vi "Type Definition Folder Name--constant.vi"() -> (3 "Type Definition Folder Name":string)   [LabVIEW 2026]
doc: "This constant defines the name of the type definitions folder on the main project directory."
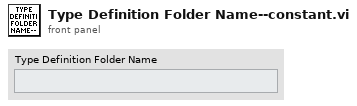
[diagram p1: front panel]
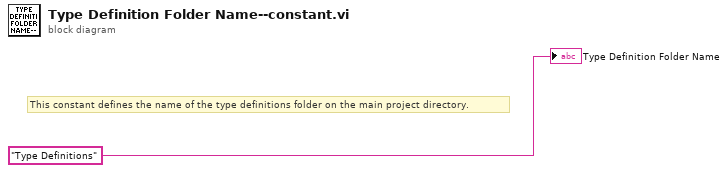
[diagram p0: block diagram]
diagram:
  # "This constant defines the name of the type definitions folder on the main project directory."
  "Type Definition Folder Name" <- "Type Definitions"
